vi "VIH Platform - Windows - Find Executable Associated with a File.vi"(6 "cmd (run)":enum16{"run", "check"}(ring), 8 "error in":errorcluster, 9 "default directory":path, 11 "Document path":path) -> (0 "error out":errorcluster, 2 "ExePath":path)   [LabVIEW 2014]
doc: "::: VI Helpeks :::\nCopyright (c) 2000-2026 Konstantin Shifershteyn. All rights reserved."
panel:
  # "VI Helpeks\nCopyright (c) 2012-2026 Konstantin Shifershteyn"
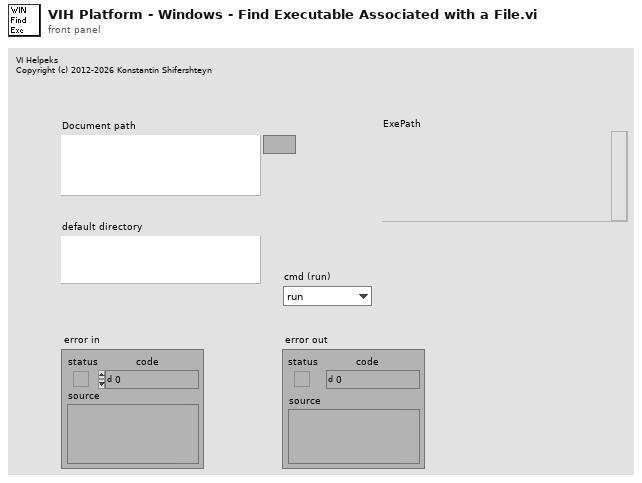
[diagram p1: front panel]
types:
  T1 = cluster{"Product Name":string, "Short Name":string, "Product Version":string, "Release Timestamp":string, "Developer":string, "Copyright":string}
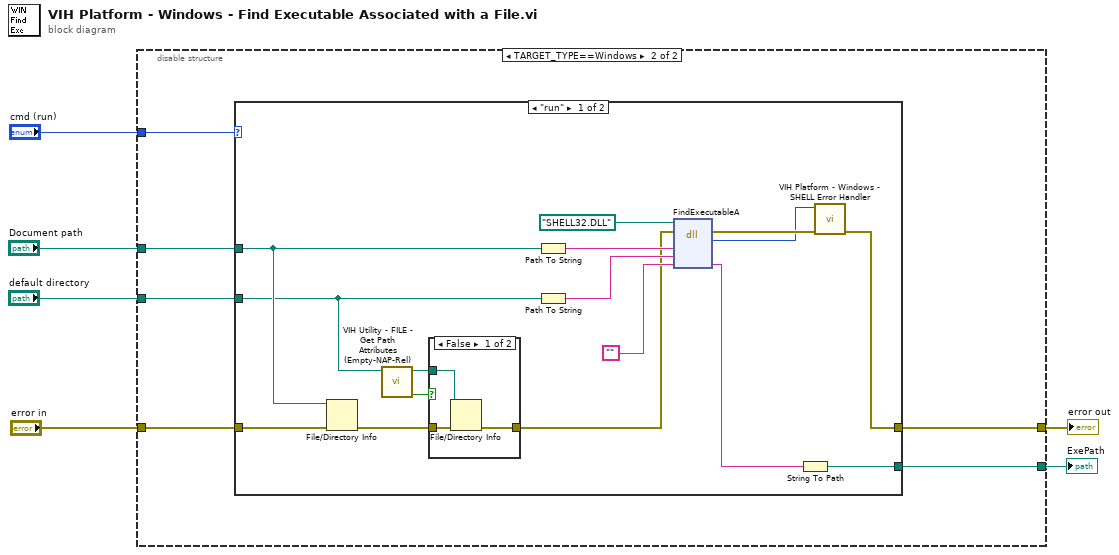
[diagram p0: block diagram]
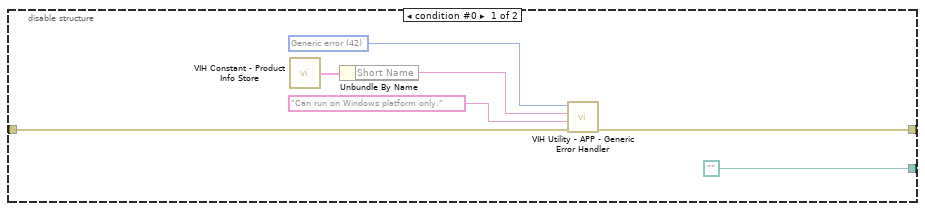
[diagram p2: hidden frame]
diagram:
  n1 = disable-structure shown="TARGET_TYPE==Windows" {
    disable-tunnel: "Document path" -> [_ w19]
    disable-tunnel: "default directory" -> [_ w18]
    disable-tunnel: "error in" -> [w12 w17]
    disable-tunnel: [w13 w16] -> w3
    disable-tunnel: "cmd (run)" -> [_ w15]
    disable-tunnel: [path "" w14] -> w1
    frame condition #0 {
      w11 = 42 items=["No error", "Argument error", "Memory is full", "Out of zone", "End of file", "File already open", "Generic file I/O error", "File not found", "File permission error", "Disk is full", "Duplicate path", "Too many files open", "System feature not enabled", "Resource file not found", "Cannot add resource", "Resource not found", "Image not found", "Image memory error", "Pen does not exist", "Config type invalid", "Config token not found", "Config parse error", "Config memory error", "Bad external code format", "Bad external code offset", "External code not present", "Null window", "Destroy window error", "Null menu", "Print aborted", "Bad print record", "Print driver error", "Windows error during printing", "Memory error during printing", "Print dialog error", "Generic print error", "Invalid device refnum", "Device not found", "Device parameter error", "Device unit error", "Cannot open device", "Device call aborted", "Generic error", "Cancelled by user", "Object ID too low", "Object ID too high", "Object not in heap", "Unknown heap", "Unknown object (invalid DefProc)", "Unknown object (DefProc not in table)", "Message out of range", "Invalid (null) method", "Unknown message", "Manager call not supported", "Bad address", "Network operation in progress", "Network operation timed out", "Connection is busy", "Network attribute not supported", "Network error", "Address in use", "System out of memory", "Connection aborted", "Connection refused", "Not connected", "Already connected", "Connection closed", "Initialization error (interapplication manager)", "Bad occurrence", "Wait on unbound occurrence handler", "Occurrence queue overflow", "Datalog type conflict", "Unused", "Unrecognized type (interapplication manager)", "Memory corrupt", "Failed to make temporary DLL", "Old CIN version", "Drag socket not found", "Failed to load drop-object", "Failed to register OLE object", "Failed to release OLE object", "Format specifier type mismatch", "Unknown format specifier", "Too few format specifiers", "Too many format specifiers", "Scan failed", "Newer CIN version", "Error converting to variant", "Runtime menu error", "Password tampered", "Variant attribute not found", "Incompatible variant data type", "Event data is not available", "Event Store is not present", "Occurrence is not found", "Event Queue is not created", "Event info is not available in the type library", "Refnum passed is NULL", "Error retrieving Class GUID", "Error retrieving CoClass GUID", "Error retrieving TypeLib GUID.", "Bad built application magic bytes.", "Specific driver is different from the specific driver associated with the Logical Name.", "There is no session opened to the class driver.", "Max Error", "MAX - Error with config objects", "MAX - Error loading configuration", "MAX - Group not supported", "Singlecast connections can not send to multicast addresses.", "Multicast connections can not send to singlecast addresses.", "Specified IP address not in multicast address range.", "Attempt to write to read-only multicast connection.", "Attempt to read from write-only multicast connection.", "The buffer used to receive a datagram was smaller than the datagram itself"]
      n2 = call "VIH Constant - Product Info Store.vi"() -> ("Product Info"=w8:T1)
      n3 = Unbundle By Name(w8) -> ("Short Name"=w7:string)
      n4 = call "VIH Utility - APP - Generic Error Handler.vi"("error in"=w12, "error reason"="Can run on Windows platform only.", "error location"=w7, "error code"=w11) -> ("error out"=w13:errorcluster)  [unwired: 6 in, 1 out]
    }
    frame condition #1 (active) {
      n5 = case shown="\"run\"" w15 {
        tunnel: w19 -> [w25 _]
        tunnel: w18 -> [w21 _]
        tunnel: [w27 w40] -> w16
        tunnel: w17 -> [w26 w40]
        tunnel: [w30 _] -> w14
        frame "run" {
          n6 = File/Directory Info(path=w25, error in=w26) -> (error out=w24:errorcluster)  [unwired: 6 out]
          n7 = call "VIH Utility - FILE - Get Path Attributes (Empty-NAP-Rel).vi"("Path"=w21) -> ("Not A Path or Empty path"=w22:bool, "dup Path"=w20:path)  [unwired: 6 in, 3 out]
          n8 = case shown="False" w22 {
            tunnel: w24 -> [w38 w39]
            tunnel: [w37 w39] -> w23
            tunnel: w20 -> [w36 _]
            frame False {
              n9 = File/Directory Info(path=w36, error in=w38) -> (error out=w37:errorcluster)  [unwired: 6 out]
            }
            frame True {
            }
          }
          n10 = Path To String(path=w25) -> (string=w34:string)
          n11 = Path To String(path=w21) -> (string=w32:string)
          n12 = dll-call lib="SHELL32.DLL" fn="FindExecutableA"(path in=path "SHELL32.DLL", error in=w23, "File"=w34, "DefaultDir"=w32, "ExePath"="") -> (error out=w29:errorcluster, "return value"=w28:i32, "ExePath"=w31:string)  [unwired: 3 in, 1 out]
          n13 = String To Path(string=w31) -> (path=w30:path)
          n14 = call "VIH Platform - Windows - SHELL Error Handler.vi"("error in"=w29, "SHELL Error Code"=w28) -> ("error out"=w27:errorcluster)  [unwired: 9 in]
        }
        frame "check" {
        }
      }
    }
  }
  "error out" <- w3
  "ExePath" <- w1
